vi "test1-LocalExternalStatusRegistration.vi"(8 "error in (no error)":errorcluster, 11 "TestCase in":refnum<class "testcase-CSMBroadcast.lvclass">) -> (0 "error out":errorcluster, 3 "TestCase out":refnum<class "testcase-CSMBroadcast.lvclass">)   [LabVIEW 2017, in "testcase-CSMBroadcast.lvclass"]
uses:
  testcase-CSMBroadcast.lvclass
  0b17d103-e67b-41be-a9eb-a2ee1311ff1f.vi
  5999693e-4f8a-4b34-ae87-f34dff5771be.vi
  de2dcf32-e0f3-4ce3-ae15-c78c2a65fbc0.vi
  52a2a10a-a04b-4bad-8df4-e1eb944f47cc.vi
  826f03dd-b4b5-4c6b-9085-8edf6da4f43b.vi
  src/user.lib/_NEVSTOP/Communicable State Machine(CSM)/AdvanceAPI/CSM - Revert Arguments-Safe String.vi
  src/user.lib/_NEVSTOP/Communicable State Machine(CSM)/_Shared/Trim Single-line Text.vi
  src/user.lib/_NEVSTOP/Communicable State Machine(CSM)/AdvanceAPI/CSM - Make String Arguments Safe.vi
  src/user.lib/_NEVSTOP/Communicable State Machine(CSM)/AdvanceAPI/CSM - Break Down Multiple States String.vi
  src/user.lib/_NEVSTOP/Communicable State Machine(CSM)/AdvanceAPI/CSM - Keywords.vi
  src/user.lib/_NEVSTOP/Communicable State Machine(CSM)/_Polymophic/CSM - Replace Marks in Messages.vi
  src/user.lib/_NEVSTOP/Communicable State Machine(CSM)/AdvanceAPI/CSM - Get Module Attribute.vi
  <vilib>/addons/_JKI Toolkits/VI Tester/TestCase.llb/TestCase.lvclass
  src/user.lib/_NEVSTOP/Communicable State Machine(CSM)/Communicable State Machine.lvlib
  C:/Program Files (x86)/National Instruments/LabVIEW 2017/vi.lib/addons/_JKI Toolkits/VI Tester/TestCase.llb/TestCase.lvclass
panel:
  out "One-Shot Unregistrations":string
  out "One-Shot Registrations":string
  out "LoopCount 2":i32
  out "State History":string
  out "LoopCount":i32
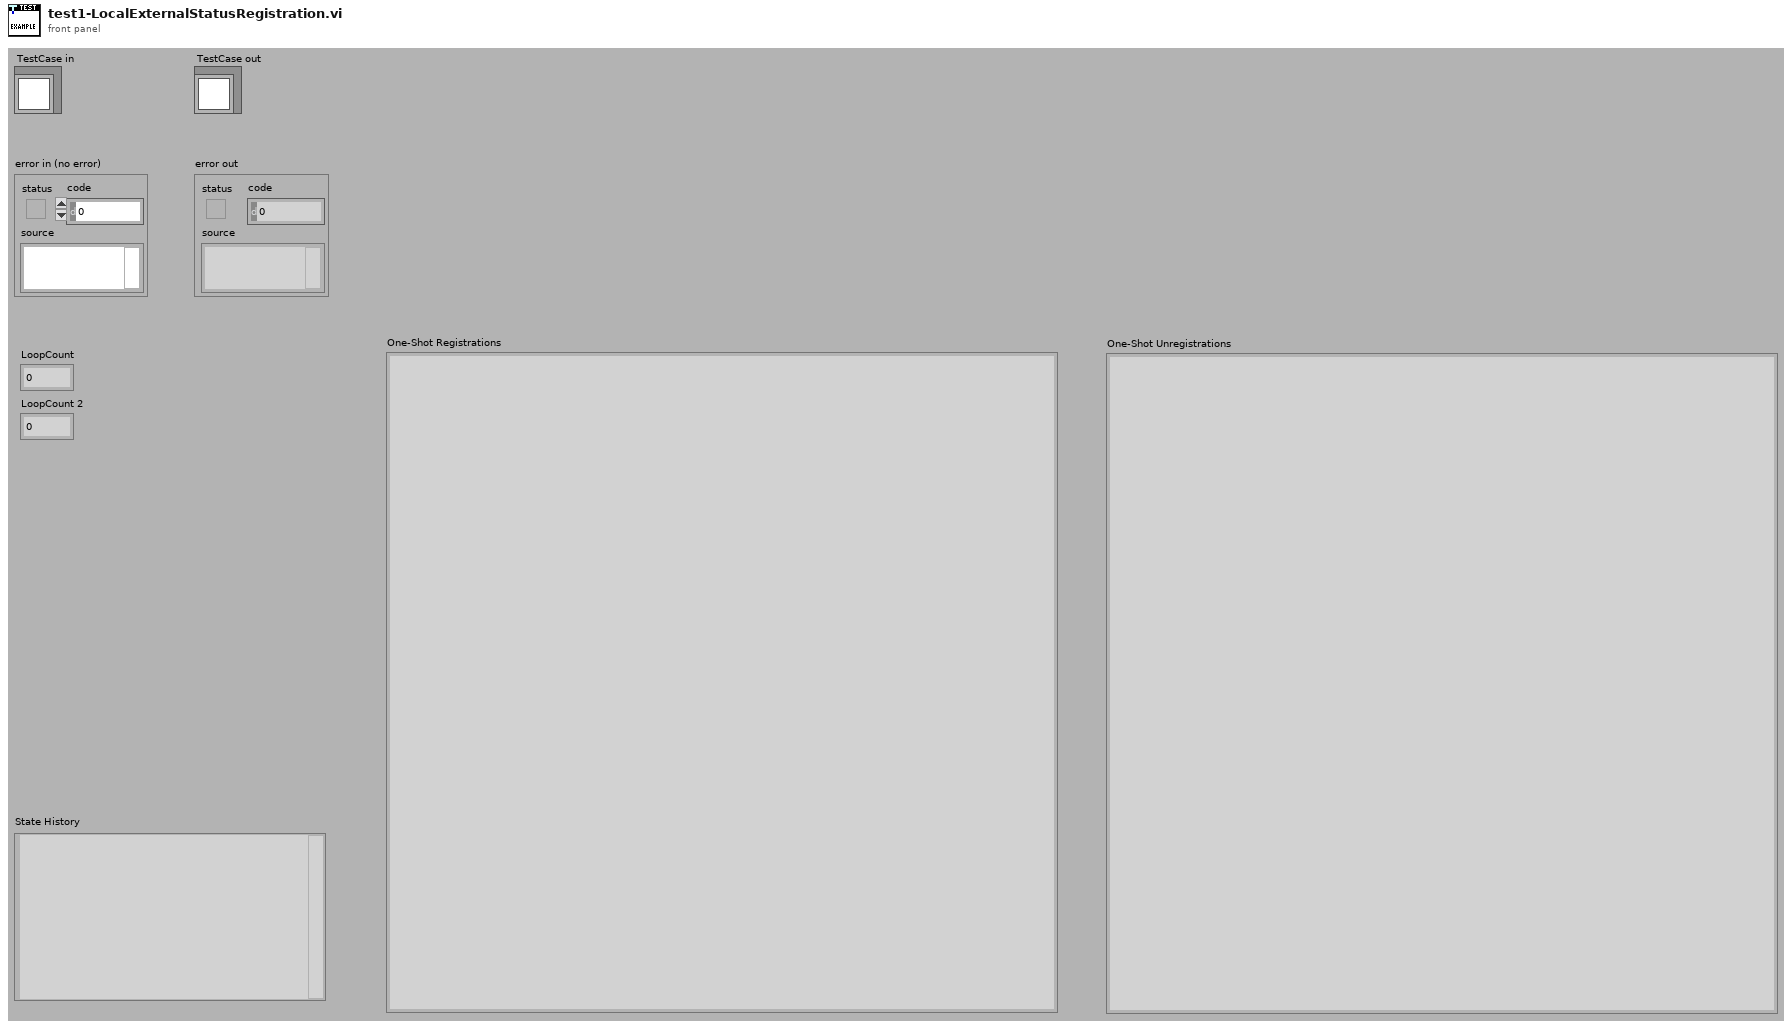
[diagram p1: front panel]
types:
  T1 = enum32{"Invalid", "Standard", "Closed", "Hidden", "Minimized", "Maximized"}
  T2 = enum32{"invalid app kind", "Development System", "Run Time System", "Student Edition", "Embedded LabVIEW", "Evaluation", "Custom"}
  T3 = typedef "Communicable State Machine.lvlib/_CSM_Response Source Message.ctl" = cluster{"‘State":string, "’Arguments":string, "’Error":errorcluster}
  T4 = cluster{"Current VI Reference":refnum<vi>, "Close Panel on Exit?":bool}
  T5 = cluster{"Core":cluster{"Current VI Reference":refnum<vi>, "Close Panel on Exit?":bool}, "Your Boolean data":bool, "Your string data":string}
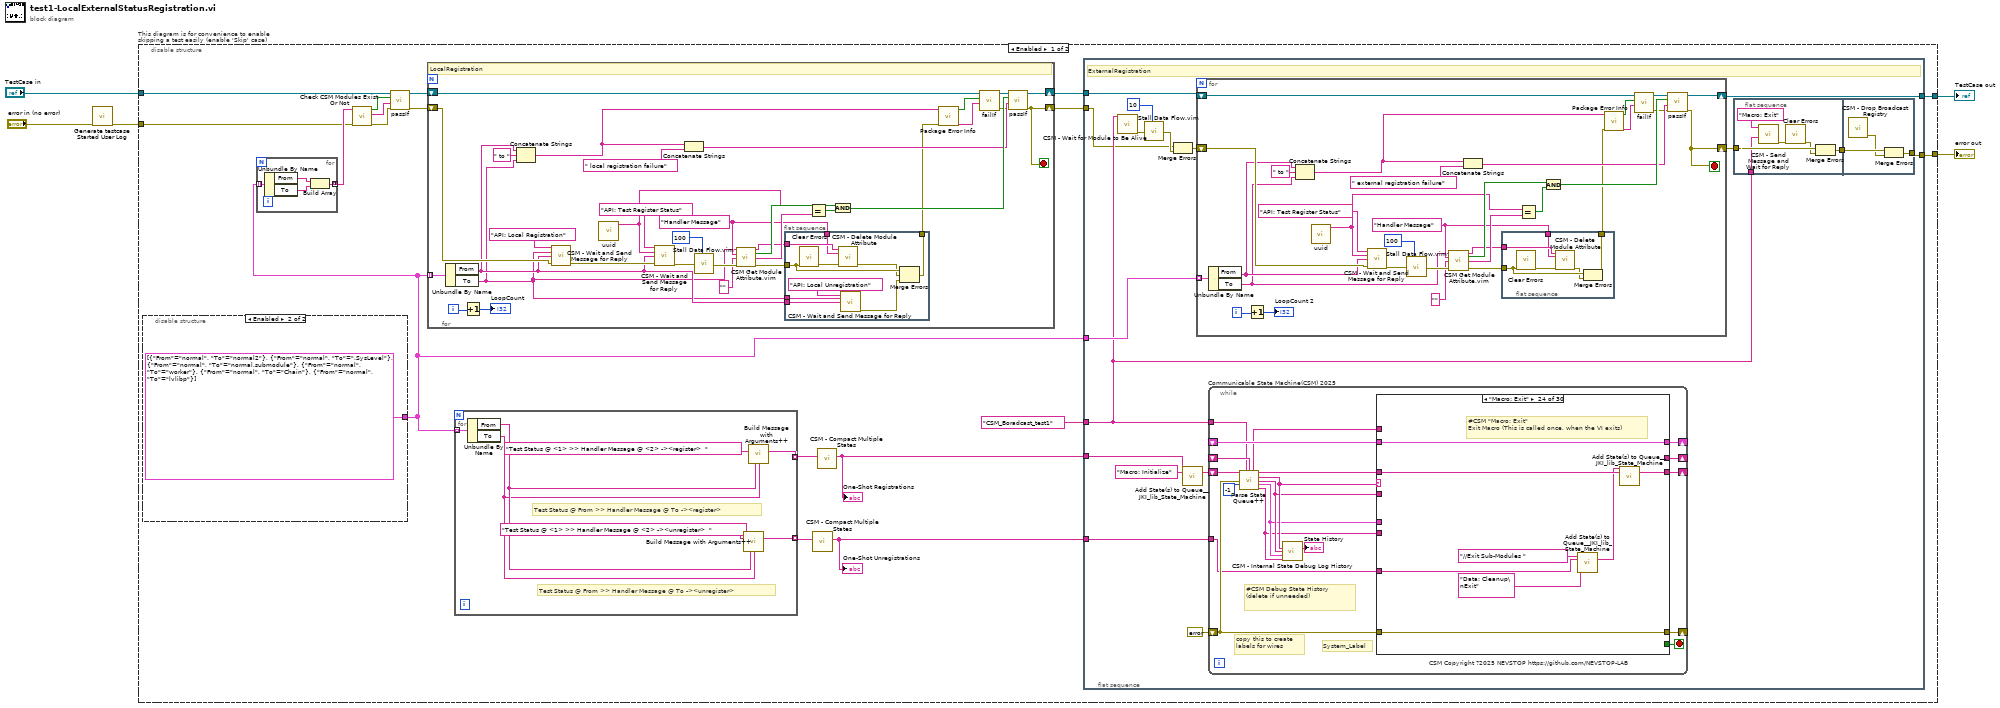
[diagram p0: block diagram]
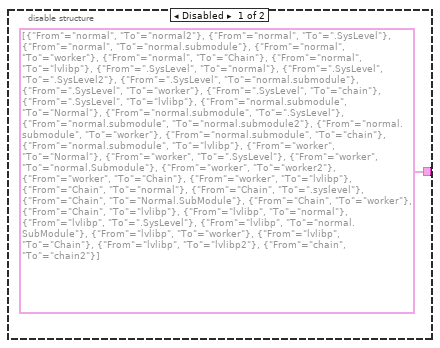
[diagram p2: hidden frame]
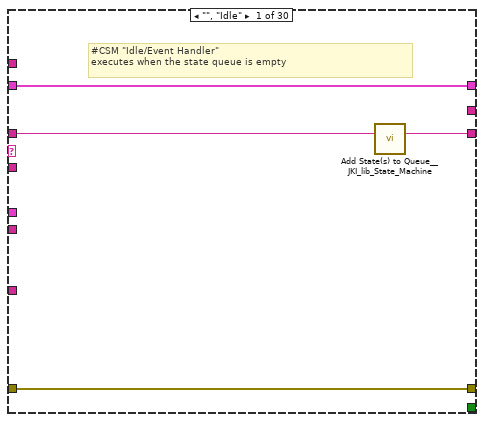
[diagram p3: hidden frame]
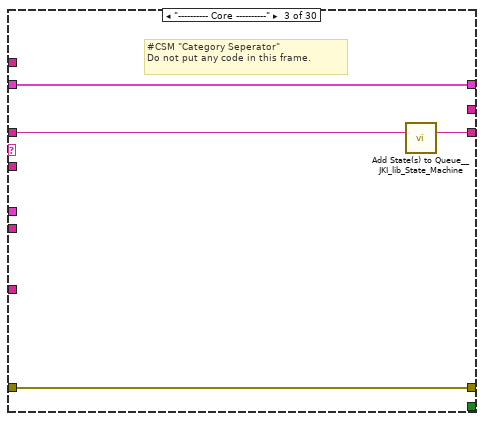
[diagram p5: hidden frame]
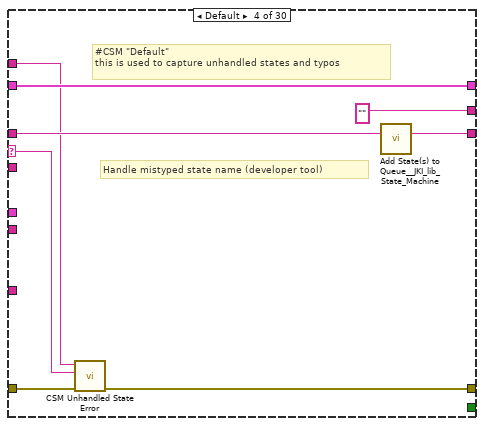
[diagram p6: hidden frame]
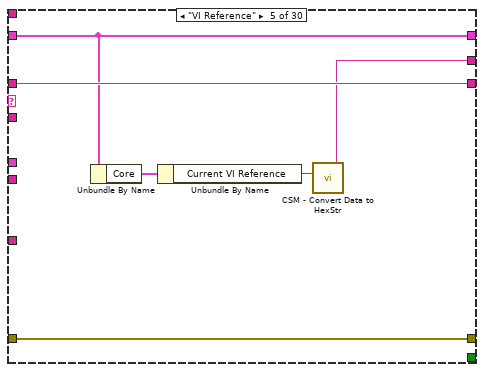
[diagram p7: hidden frame]
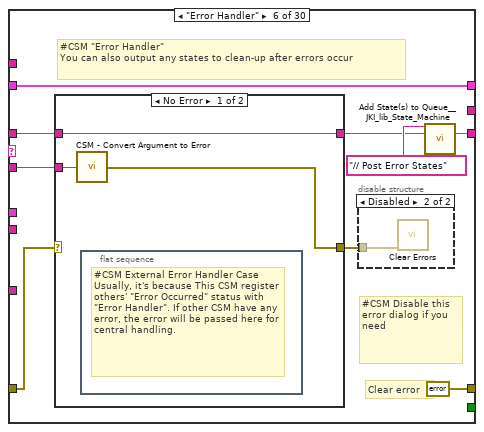
[diagram p8: hidden frame]
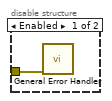
[diagram p9: hidden frame]
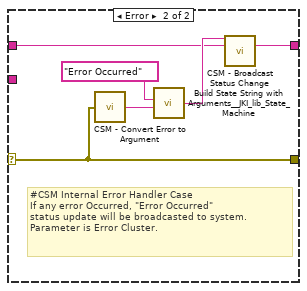
[diagram p10: hidden frame]
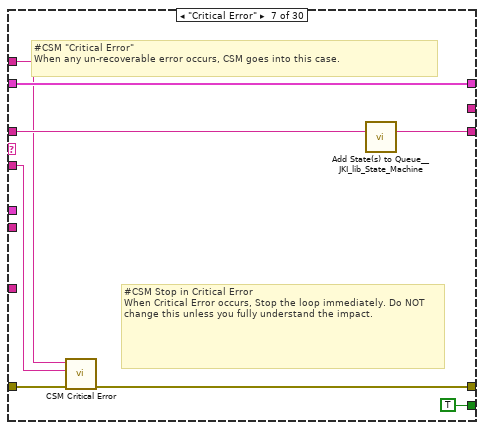
[diagram p11: hidden frame]
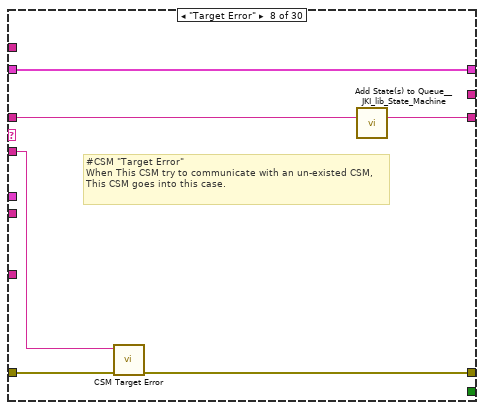
[diagram p12: hidden frame]
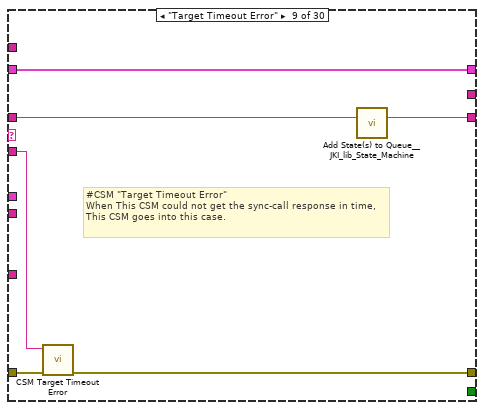
[diagram p13: hidden frame]
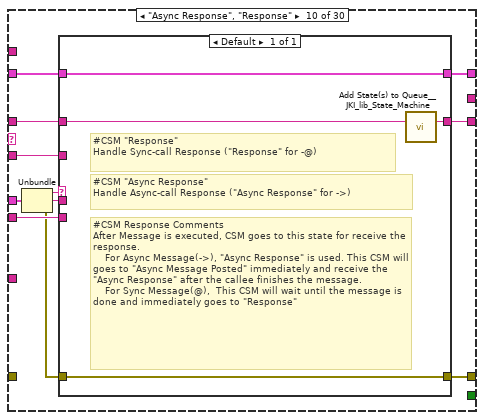
[diagram p14: hidden frame]
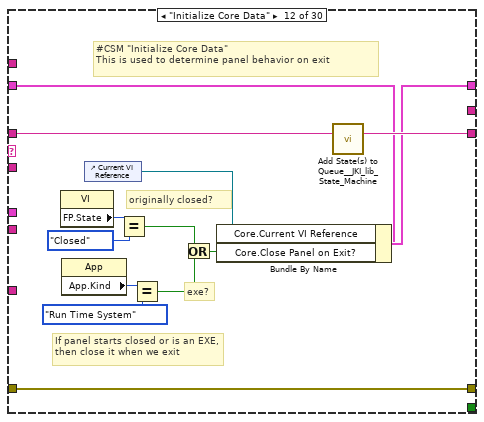
[diagram p16: hidden frame]
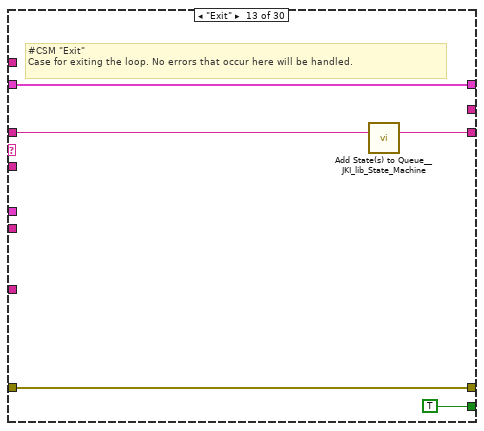
[diagram p17: hidden frame]
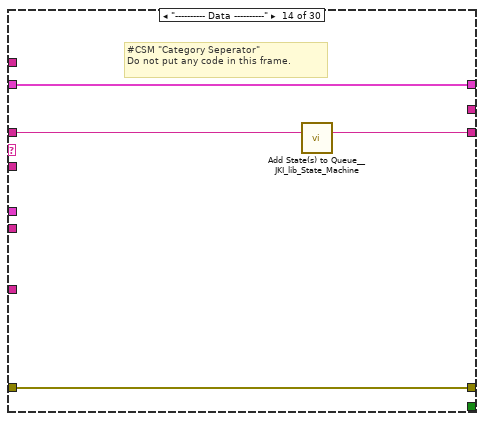
[diagram p18: hidden frame]
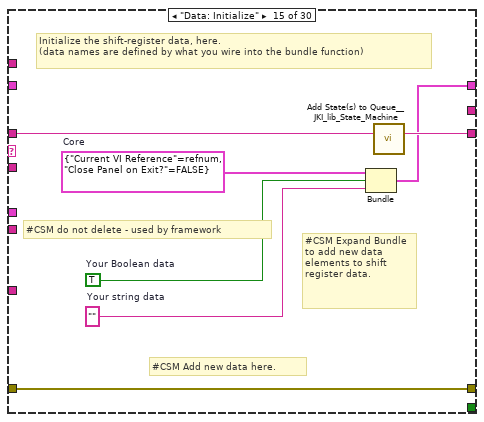
[diagram p19: hidden frame]
diagram:
  n1 = call "Generate testcase Started User Log.vi"("Error In"="error in (no error)") -> ("error out"=w1:errorcluster)  [unwired: 10 in]
  n2 = disable-structure "This diagram is for convenience to enable skipping a test easily (enable 'Skip' case)" shown="Enabled" {
    disable-tunnel: "TestCase in" -> [w11 w423]
    disable-tunnel: [w22 w421] -> w2
    disable-tunnel: [w16 w422] -> w4
    disable-tunnel: w1 -> [w9 w420]
    frame Enabled {
      n3 = disable-structure shown="Enabled" {
        disable-tunnel: [cluster{"From":string, "To":string}[] [{"From"="normal", "To"="normal2"}, {"From"="normal", "To"=".SysLevel"}, {"From"="normal", "To"="normal.submodule"}, {"From"="normal", "To"="worker"}, {"From"="normal", "To"="Chain"}, {"From"="normal", "To"="lvlibp"}, {"From"=".SysLevel", "To"="normal"}, {"From"=".SysLevel", "To"=".SysLevel2"}, {"From"=".SysLevel", "To"="normal.submodule"}, {"From"=".SysLevel", "To"="worker"}, {"From"=".SysLevel", "To"="chain"}, {"From"=".SysLevel", "To"="lvlibp"}, {"From"="normal.submodule", "To"="Normal"}, {"From"="normal.submodule", "To"=".SysLevel"}, {"From"="normal.submodule", "To"="normal.submodule2"}, {"From"="normal.submodule", "To"="worker"}, {"From"="normal.submodule", "To"="chain"}, {"From"="normal.submodule", "To"="lvlibp"}, {"From"="worker", "To"="Normal"}, {"From"="worker", "To"=".SysLevel"}, {"From"="worker", "To"="normal.Submodule"}, {"From"="worker", "To"="worker2"}, {"From"="worker", "To"="Chain"}, {"From"="worker", "To"="lvlibp"}, {"From"="Chain", "To"="normal"}, {"From"="Chain", "To"=".syslevel"}, {"From"="Chain", "To"="Normal.SubModule"}, {"From"="Chain", "To"="worker"}, {"From"="Chain", "To"="lvlibp"}, {"From"="lvlibp", "To"="normal"}, {"From"="lvlibp", "To"=".SysLevel"}, {"From"="lvlibp", "To"="normal.SubModule"}, {"From"="lvlibp", "To"="worker"}, {"From"="lvlibp", "To"="Chain"}, {"From"="lvlibp", "To"="lvlibp2"}, {"From"="chain", "To"="chain2"}] cluster{"From":string, "To":string}[] [{"From"="normal", "To"="normal2"}, {"From"="normal", "To"=".SysLevel"}, {"From"="normal", "To"="normal.submodule"}, {"From"="normal", "To"="worker"}, {"From"="normal", "To"="Chain"}, {"From"="normal", "To"="lvlibp"}]] -> w6
        frame Disabled {
        }
        frame Enabled {
        }
      }
      n4 = for {
        tunnel: w6 -> [w29] mode=indexing
        tunnel: [w26] -> w14 mode=concatenating
        n5 = Unbundle By Name(w29) -> ("From"=w28:string, "To"=w27:string)
        n6 = Build Array(w28, w27) -> (w26:string[])
      }
      n7 = call "Check CSM Modules Exist Or Not.vi"("error in"=w9, "CSM names in"=w14) -> ("error out"=w12:errorcluster, "Debug string"=w13:string, "All Modules Exist?"=w15:bool)  [unwired: 7 in]
      n8 = call-dynamic "passIf.vi"("error in (no error)"=w12, "message (\"\")"=w13, "pass"=w15, "TestCase in"=w11) -> ("error out"=w8:errorcluster, "TestCase out"=w10:refnum<class "testcase-CSMBroadcast.lvclass">)  [unwired: 6 in]
      n9 = for {
        shift-right: [w42] -> w21
        shift-left: w8 -> [w43]
        shift-right: [w49] -> w23
        shift-left: w10 -> [w34]
        tunnel: w6 -> [w60] mode=indexing
        i -> [w62]
        stop <- w42 stop-if-true
        w44 = "Handler Message" ("To")
        # "LocalRegistration"
        n10 = Unbundle By Name(w60) -> ("From"=w40:string, "To"=w39:string)
        n11 = Increment(x=w62) -> (x+1=→"LoopCount":i32)
        n12 = Concatenate Strings(w40, " to " ("string"), w39) -> (w30:string)
        n13 = call "CSM - Wait and Send Message for Reply.vi"("State"="API: Local Registration", "Arguments (\"\")"=w39, "Target Module"=w40, "Error In (No Error)"=w43) -> ("error out"=w57:errorcluster)  [unwired: 8 in, 3 out]
        n14 = call "uuid.vi"() -> ("UUID"=w51:string)  [unwired: 11 in]
        n15 = call "CSM - Wait and Send Message for Reply.vi"("State"="API: Test Register Status", "Arguments (\"\")"=w51, "Target Module"=w40, "Error In (No Error)"=w57) -> ("error out"=w56:errorcluster)  [unwired: 8 in, 3 out]
        n16 = Concatenate Strings(w30, " local registration failure" ("string")) -> (w37:string)
        n17 = call "Stall Data Flow.vim"("value in"=w56, "milliseconds to wait"=u32 100) -> ("value out"=w54:errorcluster)  [unwired: 1 out]
        n18 = call "CSM Get Module Attribute.vim"("CSM Name"=w39, "Attribute"=w44, "Default Value (Empty Variant)"="", "Error In"=w54) -> ("CSM Name (Dup)"=w45:string, "Found"=w53:bool, "Value"=w50:string, "error out"=w46:errorcluster)  [unwired: 7 in, 1 out]
        n19 = flat-sequence {
          tunnel: w46 -> [w66]
          tunnel: w45 -> [w71]
          tunnel: w44 -> [w70]
          tunnel: w39 -> [w68]
          tunnel: w40 -> [w67]
          tunnel: [w63] -> w31
          frame #0 {
            n20 = call <vilib>:"Clear Errors.vi"("error in (no error)"=w66) -> ("error out"=w72:errorcluster)  [unwired: 5 in, 1 out]
            n21 = call "CSM - Delete Module Attribute.vi"("CSM Name"=w71, "Attribute"=w70, "Error In"=w72) -> ("error out"=w65:errorcluster)  [unwired: 9 in, 3 out]
            n22 = call "CSM - Wait and Send Message for Reply.vi"("State"="API: Local Unregistration", "Arguments (\"\")"=w68, "Target Module"=w67) -> ("error out"=w64:errorcluster)  [unwired: 9 in, 3 out]
            n23 = Merge Errors(w66, w65, w64) -> (w63:errorcluster)
          }
        }
        n24 = Equal?(x=w51, y=w50) -> (x = y?=w48:bool)
        n25 = And(x=w53, y=w48) -> (x .and. y?=w47:bool)
        n26 = call "Package Error Info.vi"("error in"=w31, "String in"=w30) -> ("packed error info out"=w35:string, "error status"=w36:bool)  [unwired: 8 in]
        n27 = call-dynamic "failIf.vi"("message (\"\")"=w35, "fail"=w36, "TestCase in"=w34) -> ("error out"=w32:errorcluster, "TestCase out"=w33:refnum<class "testcase-CSMBroadcast.lvclass">)  [unwired: 7 in]
        n28 = call-dynamic "passIf.vi"("error in (no error)"=w32, "message (\"\")"=w37, "pass"=w47, "TestCase in"=w33) -> ("error out"=w42:errorcluster, "TestCase out"=w49:refnum<class "testcase-CSMBroadcast.lvclass">)  [unwired: 6 in]
      }
      n29 = for {
        tunnel: w6 -> [w78] mode=indexing
        tunnel: [w77] -> w20 mode=indexing
        tunnel: [w73] -> w18 mode=indexing
        # "Test Status @ From >> Handler Message @ To -><unregister>"
        # "Test Status @ From >> Handler Message @ To -><register>"
        n30 = Unbundle By Name(w78) -> ("From"=w75:string, "To"=w74:string)
        n31 = call-poly "Build Message with Arguments++.vi"("States With Replace Token"="Test Status @ <1> >> Handler Message @ <2> -><unregister>  " ("State"), "<1>"=w75, "<2>"=w74) -> ("States"=w73:string)  [unwired: 12 in]
        n32 = call-poly "Build Message with Arguments++.vi"("States With Replace Token"="Test Status @ <1> >> Handler Message @ <2> -><register>  " ("State"), "<1>"=w75, "<2>"=w74) -> ("States"=w77:string)  [unwired: 12 in]
      }
      n33 = call "CSM - Compact Multiple States.vi"("Multiple States"=w18) -> ("States"=w17:string)  [unwired: 9 in]
      "One-Shot Unregistrations" <- w17
      n34 = call "CSM - Compact Multiple States.vi"("Multiple States"=w20) -> ("States"=w19:string)  [unwired: 9 in]
      "One-Shot Registrations" <- w19
      n35 = flat-sequence {
        tunnel: w23 -> [w93]
        tunnel: [w92] -> w22
        tunnel: w21 -> [w80]
        tunnel: w6 -> [w91]
        tunnel: w19 -> [w90]
        tunnel: w17 -> [w87]
        tunnel: [w85] -> w16
        tunnel: "CSM_Boradcast_test1" ("Name (\"\" to Use UUID)") -> [w84]
        frame #0 {
          # "ExternalRegistration"
          n36 = call "CSM - Wait for Module to Be Alive.vi"("CSM Name"=w84) -> ("error out"=w83:errorcluster)  [unwired: 12 in, 2 out]
          n37 = call "Stall Data Flow.vim"("value in"=w83, "milliseconds to wait"=u32 10) -> ("value out"=w82:errorcluster)  [unwired: 1 out]
          n38 = Merge Errors(w80, w82) -> (w88:errorcluster)
          n39 = call <vilib>:"Add State(s) to Queue__JKI_lib_State_Machine.vi"("State(s) in Front (\"\")"=w90, "State(s) in (\"\")"="Macro: Initialize" ("Init State(\"Macro: Initialize\")")) -> ("States Out"=w94:string)  [unwired: 13 in]
          n40 = for {
            shift-right: [w118] -> w89
            shift-left: w88 -> [w119]
            shift-right: [w125] -> w92
            shift-left: w93 -> [w110]
            tunnel: w91 -> [w134] mode=indexing
            i -> [w136]
            stop <- w118 stop-if-true
            w120 = "Handler Message" ("To")
            n41 = Unbundle By Name(w134) -> ("From"=w115:string, "To"=w114:string)
            n42 = Increment(x=w136) -> (x+1=→"LoopCount 2":i32)
            n43 = Concatenate Strings(w115, " to " ("string"), w114) -> (w106:string)
            n44 = call "uuid.vi"() -> ("UUID"=w127:string)  [unwired: 11 in]
            n45 = call "CSM - Wait and Send Message for Reply.vi"("State"="API: Test Register Status", "Arguments (\"\")"=w127, "Target Module"=w115, "Error In (No Error)"=w119) -> ("error out"=w132:errorcluster)  [unwired: 8 in, 3 out]
            n46 = call "Stall Data Flow.vim"("value in"=w132, "milliseconds to wait"=u32 100) -> ("value out"=w130:errorcluster)  [unwired: 1 out]
            n47 = call "CSM Get Module Attribute.vim"("CSM Name"=w114, "Attribute"=w120, "Default Value (Empty Variant)"="", "Error In"=w130) -> ("CSM Name (Dup)"=w121:string, "Found"=w129:bool, "Value"=w126:string, "error out"=w122:errorcluster)  [unwired: 7 in, 1 out]
            n48 = Concatenate Strings(w106, " external registration failure" ("string")) -> (w113:string)
            n49 = flat-sequence {
              tunnel: w122 -> [w139]
              tunnel: w121 -> [w141]
              tunnel: w120 -> [w140]
              tunnel: [w137] -> w107
              frame #0 {
                n50 = call <vilib>:"Clear Errors.vi"("error in (no error)"=w139) -> ("error out"=w142:errorcluster)  [unwired: 5 in, 1 out]
                n51 = call "CSM - Delete Module Attribute.vi"("CSM Name"=w141, "Attribute"=w140, "Error In"=w142) -> ("error out"=w138:errorcluster)  [unwired: 9 in, 3 out]
                n52 = Merge Errors(w139, w138) -> (w137:errorcluster)
              }
            }
            n53 = Equal?(x=w127, y=w126) -> (x = y?=w124:bool)
            n54 = And(x=w129, y=w124) -> (x .and. y?=w123:bool)
            n55 = call "Package Error Info.vi"("error in"=w107, "String in"=w106) -> ("packed error info out"=w111:string, "error status"=w112:bool)  [unwired: 8 in]
            n56 = call-dynamic "failIf.vi"("message (\"\")"=w111, "fail"=w112, "TestCase in"=w110) -> ("error out"=w108:errorcluster, "TestCase out"=w109:refnum<class "testcase-CSMBroadcast.lvclass">)  [unwired: 7 in]
            n57 = call-dynamic "passIf.vi"("error in (no error)"=w108, "message (\"\")"=w113, "pass"=w123, "TestCase in"=w109) -> ("error out"=w118:errorcluster, "TestCase out"=w125:refnum<class "testcase-CSMBroadcast.lvclass">)  [unwired: 6 in]
          }
          n58 = while "Communicable State Machine(CSM) 2025" {
            shift-right: [w156] -> _
            shift-left: _ -> [w155]
            shift-right: [w159] -> _
            shift-left: errorcluster {"status"=FALSE, "code"=0, "source"=""} ("error out") -> [w154]
            shift-right: [w158] -> _
            shift-left: w94 -> [w160]
            shift-right: [w153] -> _
            shift-left: _ -> [w147]
            tunnel: w87 -> [w144]
            tunnel: w84 -> [w143]
            stop <- w157 stop-if-true
            # "#CSM Debug State History\n(delete if unneeded)"
            # "copy this to create labels for wires"
            # "System_Label"
            # "CSM Copyright ?2025 NEVSTOP https://github.com/NEVSTOP-LAB"
            n59 = call "Parse State Queue++.vi"("State Queue"=w160, "Name (\"\" to Use UUID)"=w143, "Response Arguments"=w147, "Previous Error"=w154, "Dequeue (1 ms)"=-1 ("Timeout")) -> ("Name Used"=w148:string, "Remaining States"=w161:string, "Current State"=w152:string, "Arguments"=w151:string, "Additional Information"=w150:T3, "Source CSM"=w149:string)  [unwired: 5 in]
            n60 = call "CSM - Internal State Debug Log History.vi"("State"=w152, "Arguments (\"\")"=w151, ">> Response Source Message >>"=w150, "Source (\"\")"=w149) -> ("Debug Log"=→"State History":string)  [unwired: 11 in]
            n61 = case shown="\"Macro: Exit\"" w152 {
              selector: w152 -> [_ _ _ w175 _ _ _ _ _ _ _ _ _ _ _ _ _ _ _ _ _ _ _ _ _ _ _ _ _ _]
              tunnel: w161 -> [w162 w167 w172 w179 w185 w191 w212 w218 w224 w232 w243 w257 w262 w266 w273 w275 w282 w286 w290 w296 w311 w380 w385 w393 w395 w399 w404 w411 w415 w419]
              tunnel: w151 -> [_ _ _ _ _ w190 w208 w217 w222 w231 _ _ _ _ _ _ _ _ _ w291 w305 _ _ _ _ _ w402 _ _ _]
              tunnel: w155 -> [w163 w166 w169 w177 w184 w194 w213 w219 w225 w234 w242 w250 w260 w263 _ w274 w277 w283 w288 w294 w307 w377 w382 w390 w394 w398 w403 w408 w412 w416]
              tunnel: [w164 w168 w170 w173 w186 errorcluster {"status"=FALSE, "code"=0, "source"=""} ("error out") w209 w215 w221 w237 w244 w254 w259 w264 w270 w276 w278 w284 w287 w292 w308 w378 w383 w391 w396 w400 w405 w409 w413 w417] -> w159
              tunnel: w154 -> [w164 w168 w170 w180 w186 w192 w214 w216 w223 _ w244 w254 w259 w264 w270 w276 w279 w284 w287 w293 w309 w378 w383 w391 w396 w400 w405 w409 w413 w417]
              tunnel: [w165 w167 w171 w178 w185 w187 w211 w220 w226 w233 w243 w256 w261 w265 w272 w275 w281 w285 w289 w295 w310 w379 w384 w392 w395 w399 w404 w410 w414 w418] -> w158
              tunnel: [_ _ _ _ _ _ TRUE _ _ _ _ _ TRUE _ _ _ _ _ _ _ _ _ _ _ _ _ _ _ _ _] -> w157
              tunnel: [w163 w166 w169 w177 w184 w194 w213 w219 w225 w235 w242 w255 w260 w263 w271 w274 w277 w283 w288 w294 w307 w377 w382 w390 w394 w398 w403 w408 w412 w416] -> w156
              tunnel: w149 -> [_ _ _ _ _ _ _ _ _ w229 _ _ _ _ _ _ _ _ _ _ _ _ _ _ _ _ _ _ _ _]
              tunnel: w150 -> [_ _ _ _ _ _ _ _ _ w236 _ _ _ _ _ _ _ _ _ _ _ _ _ _ _ _ _ _ _ _]
              tunnel: [_ _ _ "" w181 _ _ _ _ _ _ _ _ _ _ _ _ _ _ _ _ _ _ _ _ "API1 Response" w401 _ _ _] -> w153
              tunnel: w148 -> [_ _ _ w174 _ _ w207 _ _ _ _ _ _ _ _ _ _ _ _ _ _ _ _ _ _ _ _ _ _ _]
              tunnel: w144 -> [_ _ _ _ _ _ _ _ _ _ _ _ _ _ _ _ _ _ _ _ _ _ _ w386 _ _ _ _ _ _]
              frame "", "Idle" {
                # "#CSM \"Idle/Event Handler\"\nexecutes when the state queue is empty"
                n62 = call <vilib>:"Add State(s) to Queue__JKI_lib_State_Machine.vi"("State(s) in (\"\")"=w162) -> ("States Out"=w165:string)  [unwired: 14 in]
              }
              frame "CSM Documentation" {
                # "#CSM README FIRST\n\nCommunicable State Machine(CSM) is a LabVIEW application framework that builds upon JKI State Machine(JKISM). It follows the pattern of JKISM and extends the keywords to describe message communication between modules, including concepts such as Sync-Message, Async-Message, Subscription/Unsubscription of status - essential elements for creating reusable code modules. For more information, please visit the CSM wiki: https://nevstop-lab.github.io/CSM-Wiki/\n\nFor instructions on JKI State Machine, visit: http://jki.net/state-machine/\nFor information about CSM, visit: https://github.com/NEVSTOP-LAB"
                # "#CSM \"Documentation\"\nCase for holding CSM Documenation"
              }
              frame "---------- Core ----------" {
                # "#CSM \"Category Seperator\"\nDo not put any code in this frame."
                n63 = call <vilib>:"Add State(s) to Queue__JKI_lib_State_Machine.vi"("State(s) in (\"\")"=w172) -> ("States Out"=w171:string)  [unwired: 14 in]
              }
              frame Default {
                # "#CSM \"Default\"\nthis is used to capture unhandled states and typos"
                # "Handle mistyped state name (developer tool)"
                n64 = call "CSM Unhandled State Error.vi"("error in (no error)"=w180, "Undefined State"=w175, "CSM Name"=w174) -> ("error out"=w173:errorcluster)  [unwired: 8 in]
                n65 = call <vilib>:"Add State(s) to Queue__JKI_lib_State_Machine.vi"("State(s) in (\"\")"=w179) -> ("States Out"=w178:string)  [unwired: 14 in]
              }
              frame "VI Reference" {
                n66 = Unbundle By Name(w184) -> ("Core"=w183:T4)
                n67 = Unbundle By Name(w183) -> ("Current VI Reference"=w182:refnum<vi>)
                n68 = call "CSM - Convert Data to HexStr.vi"("Variant"=w182) -> ("HEX String (0-9,A-F)"=w181:string)  [unwired: 8 in]
              }
              frame "Error Handler" {
                # "#CSM Disable this error dialog if you need"
                # "#CSM \"Error Handler\"\nYou can also output any states to clean-up after errors occur"
                # "Clear error"
                n69 = case shown="No Error" w192 {
                  selector: w192 -> [_ w201]
                  tunnel: [w200 w203] -> w188
                  tunnel: w191 -> [w200 w202]
                  tunnel: w190 -> [w199 _]
                  tunnel: [w198 w201] -> w193
                  frame No Error {
                    n70 = call "CSM - Convert Argument to Error.vi"("Argument"=w199) -> ("Error"=w198:errorcluster)  [unwired: 4 in]
                    n71 = flat-sequence {
                      frame #0 {
                        # "#CSM External Error Handler Case\nUsually, it's because This CSM register others' \"Error Occurred\" status with \"Error Handler\". If other CSM have any error, the error will be passed here for central handling."
                      }
                    }
                  }
                  frame Error {
                    # "#CSM Internal Error Handler Case \nIf any error Occurred, \"Error Occurred\" \nstatus update will be broadcasted to system.\nParameter is Error Cluster."
                    n72 = call "CSM - Convert Error to Argument.vi"("Error"=w201) -> ("Argument"=w205:string)  [unwired: 4 in]
                    n73 = call <vilib>:"Build State String with Arguments__JKI_lib_State_Machine.vi"("Arguments (\"\")"=w205, "State"="Error Occurred" ("Status with Arguments")) -> ("State with Arguments"=w204:string)  [unwired: 4 in]
                    n74 = call "CSM - Broadcast Status Change.vi"("Status With Arguments"=w204, "State Queue"=w202) -> ("Remaining States"=w203:string)  [unwired: 13 in]
                  }
                }
                n75 = disable-structure shown="Disabled" {
                  disable-tunnel: w193 -> [w196 w197]
                  frame Enabled {
                    n76 = call <vilib>:"General Error Handler.vi"("error in (no error)"=w196) -> ()  [unwired: 10 in, 5 out]
                  }
                  frame Disabled {
                    n77 = call <vilib>:"Clear Errors.vi"("error in (no error)"=w197) -> ()  [unwired: 5 in, 2 out]
                  }
                }
                n78 = call <vilib>:"Add State(s) to Queue__JKI_lib_State_Machine.vi"("State(s) in Front (\"\")"="// Post Error States", "State(s) in (\"\")"=w188) -> ("States Out"=w187:string)  [unwired: 13 in]
              }
              frame "Critical Error" {
                # "#CSM Stop in Critical Error\nWhen Critical Error occurs, Stop the loop immediately. Do NOT change this unless you fully understand the impact."
                # "#CSM \"Critical Error\"\nWhen any un-recoverable error occurs, CSM goes into this case."
                n79 = call "CSM Critical Error.vi"("error in (no error)"=w214, "Arugments (As Reason)"=w208, "CSM Name"=w207) -> ("error out"=w209:errorcluster)  [unwired: 8 in]
                n80 = call <vilib>:"Add State(s) to Queue__JKI_lib_State_Machine.vi"("State(s) in (\"\")"=w212) -> ("States Out"=w211:string)  [unwired: 14 in]
              }
              frame "Target Error" {
                # "#CSM \"Target Error\"\nWhen This CSM try to communicate with an un-existed CSM, This CSM goes into this case."
                n81 = call "CSM Target Error.vi"("error in (no error)"=w216, "Arguments (As CSM Name)"=w217) -> ("error out"=w215:errorcluster)  [unwired: 9 in]
                n82 = call <vilib>:"Add State(s) to Queue__JKI_lib_State_Machine.vi"("State(s) in (\"\")"=w218) -> ("States Out"=w220:string)  [unwired: 14 in]
              }
              frame "Target Timeout Error" {
                # "#CSM \"Target Timeout Error\"\nWhen This CSM could not get the sync-call response in time, This CSM goes into this case."
                n83 = call "CSM Target Timeout Error.vi"("error in (no error)"=w223, "Arguments (As CSM Name)"=w222) -> ("error out"=w221:errorcluster)  [unwired: 9 in]
                n84 = call <vilib>:"Add State(s) to Queue__JKI_lib_State_Machine.vi"("State(s) in (\"\")"=w224) -> ("States Out"=w226:string)  [unwired: 14 in]
              }
              frame "Async Response", "Response" {
                n85 = Unbundle(w236) -> ("‘State"=w230:string, "’Arguments"=w228:string, "’Error"=w227:errorcluster)
                n86 = case shown="Default" w230 {
                  tunnel: [w241] -> w237
                  tunnel: w227 -> [w241]
                  tunnel: [w240] -> w235
                  tunnel: w234 -> [w240]
                  tunnel: [w238] -> w233
                  tunnel: w232 -> [w239]
                  tunnel: w231 -> [_]
                  tunnel: w229 -> [_]
                  tunnel: w228 -> [_]
                  frame Default {
                    # "#CSM Response Comments\nAfter Message is executed, CSM goes to this state for receive the response.\n    For Async Message(->), \"Async Response\" is used. This CSM will goes to \"Async Message Posted\" immediately and receive the \"Async Response\" after the callee finishes the message.\n    For Sync Message(@),  This CSM will wait until the message is done and immediately goes to \"Response\""
                    # "#CSM \"Async Response\"\nHandle Async-call Response (\"Async Response\" for ->)"
                    # "#CSM \"Response\"\nHandle Sync-call Response (\"Response\" for -@)"
                    n87 = call <vilib>:"Add State(s) to Queue__JKI_lib_State_Machine.vi"("State(s) in (\"\")"=w239) -> ("States Out"=w238:string)  [unwired: 14 in]
                  }
                }
              }
              frame "Async Message Posted" {
                # "#CSM \"Async Message Posted\"\nAfter Async Message is posted (-> or ->| ), CSM goes to this state for post-action.\nYou can use Argument - State to tell which Async Message is called."
              }
              frame "Initialize Core Data" {
                # "#CSM \"Initialize Core Data\"\nThis is used to determine panel behavior on exit"
                # "originally closed?"
                # "exe?"
                # "If panel starts closed or is an EXE, then close it when we exit"
                n88 = property class="VI"() -> ("FP.State"=w247:T1)  [unwired: 2 in, 2 out]
                n89 = property class="App"() -> ("App.Kind"=w253:T2)  [unwired: 2 in, 2 out]
                n90 = control-ref of="Current VI Reference"() -> (w248:refnum<vi>)
                n91 = Equal?(x=w247, y=T1."Closed" ("Front Panel Window:State")) -> (x = y?=w245:bool)
                n92 = Equal?(x=w253, y=T2."Run Time System" ("Application:Kind")) -> (x = y?=w251:bool)
                n93 = Or(x=w245, y=w251) -> (x .or. y?=w249:bool)
                n94 = Bundle By Name(cluster=w250, "Core.Current VI Reference"=w248, "Core.Close Panel on Exit?"=w249) -> (w255:T5)
                n95 = call <vilib>:"Add State(s) to Queue__JKI_lib_State_Machine.vi"("State(s) in (\"\")"=w257) -> ("States Out"=w256:string)  [unwired: 14 in]
              }
              frame "Exit" {
                # "#CSM \"Exit\"\nCase for exiting the loop. No errors that occur here will be handled."
                n96 = call <vilib>:"Add State(s) to Queue__JKI_lib_State_Machine.vi"("State(s) in (\"\")"=w262) -> ("States Out"=w261:string)  [unwired: 14 in]
              }
              frame "---------- Data ----------" {
                # "#CSM \"Category Seperator\"\nDo not put any code in this frame."
                n97 = call <vilib>:"Add State(s) to Queue__JKI_lib_State_Machine.vi"("State(s) in (\"\")"=w266) -> ("States Out"=w265:string)  [unwired: 14 in]
              }
              frame "Data: Initialize" {
                w267 = T4 {"Current VI Reference"=refnum, "Close Panel on Exit?"=FALSE}  # Core
                w269 = TRUE  # Your Boolean data
                w268 = ""  # Your string data
                # "#CSM do not delete - used by framework"
                # "#CSM Expand Bundle to add new data elements to shift register data."
                # "#CSM Add new data here."
                # "Initialize the shift-register data, here.\n(data names are defined by what you wire into the bundle function)"
                n98 = Bundle("Core"=w267, "Your Boolean data"=w269, "Your string data"=w268) -> (w271:T5)  [unwired: 1 in]
                n99 = call <vilib>:"Add State(s) to Queue__JKI_lib_State_Machine.vi"("State(s) in (\"\")"=w273) -> ("States Out"=w272:string)  [unwired: 14 in]
              }
              frame "Data: Update Indicators" {
              }
              frame "Data: Cleanup" {
                # "Cleanup any data and references, here.\n(this is called automatically, by the Macro: Exit)"
                n100 = Unbundle By Name(w277) -> ("Core.Current VI Reference"=w280:refnum<vi>)
                n101 = Close Reference(reference=w280, error in (no error)=w279) -> (error out=w278:errorcluster)
                n102 = call <vilib>:"Add State(s) to Queue__JKI_lib_State_Machine.vi"("State(s) in (\"\")"=w282) -> ("States Out"=w281:string)  [unwired: 14 in]
              }
              frame "---------- UI ----------" {
                # "#CSM \"Category Seperator\"\nDo not put any code in this frame."
                n103 = call <vilib>:"Add State(s) to Queue__JKI_lib_State_Machine.vi"("State(s) in (\"\")"=w286) -> ("States Out"=w285:string)  [unwired: 14 in]
              }
              frame "UI: Initialize" {
                # "#CSM \"UI: Initialize\"\nInitialize the User Interface, here.\n(this is called automatically, by the Macro: Init)"
                n104 = call <vilib>:"Add State(s) to Queue__JKI_lib_State_Machine.vi"("State(s) in (\"\")"=w290) -> ("States Out"=w289:string)  [unwired: 14 in]
              }
              frame "UI: Cursor Set" {
                # "#CSM \"UI: Cursor Set\"\nSet and Unset Cursor Busy.\n(Usage: \"UI: Cursor Set >> Busy|Idle\")"
                # "Argument"
                n105 = disable-structure shown="TARGET_TYPE!=Windows" {
                  disable-tunnel: w293 -> [w299 w304]
                  disable-tunnel: [w298 w304] -> w292
                  disable-tunnel: w291 -> [w297 _]
                  frame condition #0 (active) {
                    n106 = case shown="\"Idle\", Default" w297 {
                      tunnel: w299 -> [w301 w303]
                      tunnel: [w300 w302] -> w298
                      frame "Idle", Default {
                        n107 = call <vilib>:"Unset Busy.vi"("error in (no error)"=w301) -> ("error out"=w300:errorcluster)  [unwired: 10 in]
                      }
                      frame "Busy" {
                        n108 = call <vilib>:"Set Busy.vi"("error in (no error)"=w303) -> ("error out"=w302:errorcluster)  [unwired: 9 in, 1 out]
                      }
                    }
                  }
                  frame condition #1 {
                  }
                }
                n109 = call <vilib>:"Add State(s) to Queue__JKI_lib_State_Machine.vi"("State(s) in (\"\")"=w296) -> ("States Out"=w295:string)  [unwired: 14 in]
              }
              frame "UI: Front Panel State" {
                # "#CSM \"UI: Front Panel State\"\nSet Front Panel Open or Closed\n(Usage: \"UI: Front Panel State >> Open|Close\")"
                # "Argument"
                n110 = Unbundle By Name(w307) -> ("Core.Current VI Reference"=w306:refnum<vi>)
                n111 = call <vilib>:"Add State(s) to Queue__JKI_lib_State_Machine.vi"("State(s) in (\"\")"=w311) -> ("States Out"=w310:string)  [unwired: 14 in]
                n112 = case shown="\"Close\", \"Closed\"" w305 {
                  tunnel: w309 -> [w317 w332 w343 w356 w369]
                  tunnel: [w319 w333 w345 w358 w371] -> w308
                  tunnel: w306 -> [w318 w330 w344 w357 w370]
                  frame "Open", "Standard", Default {
                    w312 = T1."Standard" ("State")
                    n113 = property class="VI"(reference=w318, error in=w317) -> (reference out=w315:refnum<vi>, error out=w316:errorcluster, "FP.State"=w314:T1)
                    n114 = Not Equal?(x=w314, y=w312) -> (x != y?=w313:bool)
                    n115 = case shown="True" w313 {
                      tunnel: [w323 w325] -> w319
                      tunnel: w316 -> [w322 w325]
                      tunnel: w315 -> [w321 _]
                      tunnel: w312 -> [w320 _]
                      frame True {
                        n116 = invoke class="VI" method="FP.Open"(reference=w321, error in=w322, "Activate"=TRUE, "State"=w320) -> (error out=w323:errorcluster)  [unwired: 1 in, 4 out]
                      }
                      frame False {
                      }
                    }
                  }
                  frame "Close", "Closed" {
                    n117 = property class="VI"(reference=w330, error in=w332) -> (reference out=w329:refnum<vi>, error out=w331:errorcluster, "FP.State"=w327:T1)
                    n118 = Not Equal?(x=w327, y=T1."Closed" ("Front Panel Window:State")) -> (x != y?=w326:bool)
                    n119 = case shown="False" w326 {
                      tunnel: [w334 w337] -> w333
                      tunnel: w331 -> [w334 w336]
                      tunnel: w329 -> [_ w335]
                      frame False {
                      }
                      frame True {
                        n120 = invoke class="VI" method="FP.Close"(reference=w335, error in=w336) -> (error out=w337:errorcluster)  [unwired: 1 in, 2 out]
                      }
                    }
                  }
                  frame "Hidden", "Hide" {
                    w338 = T1."Hidden" ("State")
                    n121 = property class="VI"(reference=w344, error in=w343) -> (reference out=w341:refnum<vi>, error out=w342:errorcluster, "FP.State"=w340:T1)
                    n122 = Not Equal?(x=w340, y=w338) -> (x != y?=w339:bool)
                    n123 = case shown="True" w339 {
                      tunnel: [w349 w350] -> w345
                      tunnel: w342 -> [w348 w350]
                      tunnel: w341 -> [w347 _]
                      tunnel: w338 -> [w346 _]
                      frame True {
                        n124 = invoke class="VI" method="FP.Open"(reference=w347, error in=w348, "State"=w346) -> (error out=w349:errorcluster)  [unwired: 2 in, 4 out]
                      }
                      frame False {
                      }
                    }
                  }
                  frame "Minimize", "Minimized" {
                    w351 = T1."Minimized" ("State")
                    n125 = property class="VI"(reference=w357, error in=w356) -> (reference out=w354:refnum<vi>, error out=w355:errorcluster, "FP.State"=w353:T1)
                    n126 = Not Equal?(x=w353, y=w351) -> (x != y?=w352:bool)
                    n127 = case shown="True" w352 {
                      tunnel: [w362 w363] -> w358
                      tunnel: w355 -> [w361 w363]
                      tunnel: w354 -> [w360 _]
                      tunnel: w351 -> [w359 _]
                      frame True {
                        n128 = invoke class="VI" method="FP.Open"(reference=w360, error in=w361, "State"=w359) -> (error out=w362:errorcluster)  [unwired: 2 in, 4 out]
                      }
                      frame False {
                      }
                    }
                  }
                  frame "Maximize", "Maximized" {
                    w364 = T1."Maximized" ("State")
                    n129 = property class="VI"(reference=w370, error in=w369) -> (reference out=w367:refnum<vi>, error out=w368:errorcluster, "FP.State"=w366:T1)
                    n130 = Not Equal?(x=w366, y=w364) -> (x != y?=w365:bool)
                    n131 = case shown="True" w365 {
                      tunnel: [w375 w376] -> w371
                      tunnel: w368 -> [w374 w376]
                      tunnel: w367 -> [w373 _]
                      tunnel: w364 -> [w372 _]
                      frame True {
                        n132 = invoke class="VI" method="FP.Open"(reference=w373, error in=w374, "State"=w372) -> (error out=w375:errorcluster)  [unwired: 2 in, 4 out]
                      }
                      frame False {
                      }
                    }
                  }
                }
              }
              frame "---------- Macro ----------" {
                # "#CSM \"Category Seperator\"\nDo not put any code in this frame."
                n133 = call <vilib>:"Add State(s) to Queue__JKI_lib_State_Machine.vi"("State(s) in (\"\")"=w380) -> ("States Out"=w379:string)  [unwired: 14 in]
              }
              frame "Macro: Initialize" {
                # "#CSM \"Macro: Initialize\"\nInitialization Macro (This is called once, when the VI starts)"
                n134 = call <vilib>:"Add State(s) to Queue__JKI_lib_State_Machine.vi"("State(s) in Front (\"\")"="Data: Initialize\nInitialize Core Data\nData: Update Indicators", "State(s) in (\"\")"=w385) -> ("States Out"=w384:string)  [unwired: 13 in]
              }
              frame "Macro: Exit" {
                # "#CSM \"Macro: Exit\"\nExit Macro (This is called once, when the VI exits)"
                n135 = call <vilib>:"Add State(s) to Queue__JKI_lib_State_Machine.vi"("State(s) in Front (\"\")"="//Exit Sub-Modules ", "State(s) in (\"\")"=w386, "State(s) at Back (\"\")"="Data: Cleanup\nExit") -> ("States Out"=w388:string)  [unwired: 12 in]
                n136 = call <vilib>:"Add State(s) to Queue__JKI_lib_State_Machine.vi"("State(s) in Front (\"\")"=w388, "State(s) in (\"\")"=w393) -> ("States Out"=w392:string)  [unwired: 13 in]
              }
              frame "---------- API ----------" {
                # "#CSM \"Category Seperator\"\nDo not put any code in this frame."
              }
              frame "API: API1" {
                # "#CSM API Example\nCopy/Rename this case for your own API"
                # "#CSM Response\nConnect this to return the response of your API"
                # "#CSM >> Msg/Rep's CSM >>\nIf you need to tell who triggered this state , use this string. If it's this case itself, this string is \"\"."
                # "#CSM >> Arguments >>\nDeal with the parameter if any"
              }
              frame "API: API2" {
                # "#CSM API Example\nCopy/Rename this case for your own API"
                # "unpack Hex String  to Variant\nif complex parameter is needed."
                n137 = call "CSM - Convert HexStr to Data.vi"("HEX String"=w402) -> ()  [unwired: 7 in, 2 out]
                n138 = disable-structure shown="Disabled" {
                  disable-tunnel: [w406 "API2 Response"] -> w401
                  frame Disabled {
                    # "pack variant to hexstr \nif complex response is needed."
                    # "complex Response"
                    n139 = call "CSM - Convert Data to HexStr.vi"() -> ("HEX String (0-9,A-F)"=w406:string)  [unwired: 9 in]
                  }
                  frame Enabled {
                  }
                }
              }
              frame "---------- Action ----------" {
                # "#CSM \"Category Seperator\"\nDo not put any code in this frame."
                n140 = call <vilib>:"Add State(s) to Queue__JKI_lib_State_Machine.vi"("State(s) in (\"\")"=w411) -> ("States Out"=w410:string)  [unwired: 14 in]
              }
              frame "Action: action1" {
                # "#CSM \"Internal State\"\nThis category is used for holding internal states"
                n141 = call <vilib>:"Add State(s) to Queue__JKI_lib_State_Machine.vi"("State(s) in (\"\")"=w415) -> ("States Out"=w414:string)  [unwired: 14 in]
              }
              frame "Action: action2" {
                # "#CSM \"Internal State\"\nThis category is used for holding internal states"
                n142 = call <vilib>:"Add State(s) to Queue__JKI_lib_State_Machine.vi"("State(s) in (\"\")"=w419) -> ("States Out"=w418:string)  [unwired: 14 in]
              }
            }
          }
          n143 = flat-sequence {
            tunnel: w89 -> [w101]
            tunnel: [w100] -> w86
            tunnel: w84 -> [w99]
            tunnel: w86 -> [w105]
            tunnel: [w104] -> w85
            frame #0 {
              n144 = call "CSM - Send Message and Wait for Reply.vi"("Target Module"=w99, "State"="Macro: Exit") -> ("error out"=w98:errorcluster)  [unwired: 7 in, 2 out]
              n145 = call <vilib>:"Clear Errors.vi"("error in (no error)"=w98) -> ("error out"=w97:errorcluster)  [unwired: 5 in, 1 out]
              n146 = Merge Errors(w101, w97) -> (w100:errorcluster)
            }
            frame #1 {
              n147 = call "CSM - Drop Broadcast Registry.vi"() -> ("error out"=w103:errorcluster)  [unwired: 15 in]
              n148 = Merge Errors(w105, w103) -> (w104:errorcluster)
            }
          }
        }
      }
    }
    frame Disabled {
      # "skip test result while test is under development"
      n149 = call <vilib>:"skip.vi"("error in (no error)"=w420, "TestCase in"=w423) -> ("error out"=w422:errorcluster, "TestCase out"=w421:refnum<class "testcase-CSMBroadcast.lvclass">)  [unwired: 8 in]
    }
  }
  "error out" <- w4
  "TestCase out" <- w2
